vi "Pre Launch Init.vi"(11 "DAQ Timed SPIM in":refnum<class "DAQ Timed SPIM.lvclass">) -> (0 "error out":errorcluster, 3 "DAQ Timed SPIM out":refnum<class "DAQ Timed SPIM.lvclass">)   [LabVIEW 2020, in "DAQ Timed SPIM.lvlib" / "DAQ Timed SPIM.lvclass"]
doc: "(<B>Filename</B>: Actor Framework.lvlib:Actor.lvclass:Pre Launch Init.vi)\n\nDefines behavior that occurs after the Launch Nested Actor method is invoked but before the actor's Actor Core method begins running.\n\nBy default, this method does nothing. A descendant class may override it to define behavior."
uses:
  DAQ Timed SPIM.lvclass
  <vilib>/ActorFramework/Actor/Actor.lvclass
  <resource>/objmgr/daqmx.rc
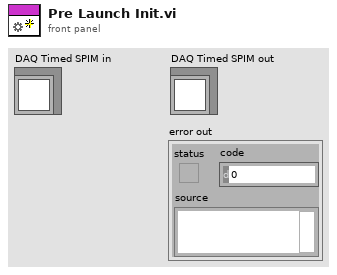
[diagram p1: front panel]
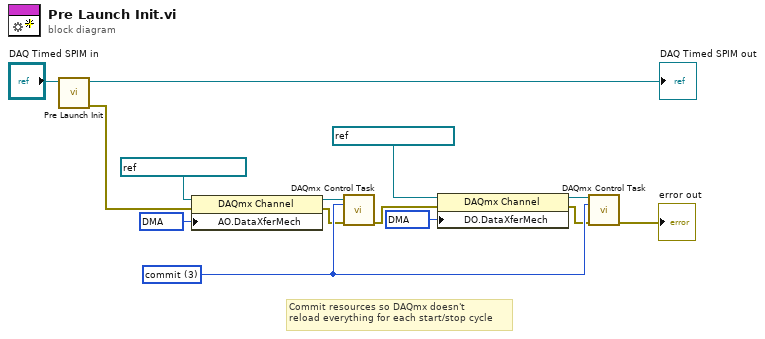
[diagram p0: block diagram]
diagram:
  w1 = 10054 items=["DMA"=10054, "Interrupts"=10204, "Programmed I/O"=10264, "USB Bulk"=12590] ("DO.DataXferMech")
  w5 = 10054 items=["DMA"=10054, "Interrupts"=10204, "Programmed I/O"=10264, "USB Bulk"=12590] ("AO.DataXferMech")
  w10 = 3 items=["verify"=2, "reserve"=4, "commit"=3, "unreserve"=5, "abort"=6] ("action")
  # "Commit resources so DAQmx doesn't\nreload everything for each start/stop cycle"
  n1 = call-parent "Pre Launch Init.vi"("Actor in"="DAQ Timed SPIM in") -> ("error out"=w9:errorcluster, "Actor out"=→"DAQ Timed SPIM out":refnum<class "DAQ Timed SPIM.lvclass">)  [unwired: 9 in]
  n2 = property class="DAQmx Channel"(reference=refnum<k21> "SPIM_Analog_Task" ("task/channels in"), error in=w9, "AO.DataXferMech"=w5) -> (reference out=w7:refnum<k21>, error out=w6:errorcluster)
  n3 = call <vilib>:"DAQmx Control Task.vi"("task/channels in"=w7, "action"=w10, "error in"=w6) -> ("error out"=w2:errorcluster)  [unwired: 11 in, 1 out]
  n4 = property class="DAQmx Channel"(reference=refnum<k21> "SPIM_Digital_Task" ("task/channels in"), error in=w2, "DO.DataXferMech"=w1) -> (reference out=w4:refnum<k21>, error out=w3:errorcluster)
  n5 = call <vilib>:"DAQmx Control Task.vi"("task/channels in"=w4, "action"=w10, "error in"=w3) -> ("error out"=→"error out":errorcluster)  [unwired: 11 in, 1 out]
